vi "FromRepo.vi"(8 "error in":errorcluster, 9 "from repo cluster":T2, 10 "repository in":refnum<class "NISE_CEF_Repository.lvclass">, 11 "engine in":refnum<class "Engine Parent Editor Node.lvclass">) -> (0 "error out":errorcluster, 2 "repository out":refnum<class "NISE_CEF_Repository.lvclass">, 3 "node":T1)   [LabVIEW 2013, in "PL Framework Configuration Tool.lvlib" / "Engine Parent Editor Node.lvclass"]
doc: "Grabs information from the Repo and stores it in the nodes."
uses:
  Engine Parent Editor Node.lvclass
  <vilib>/NI/Configuration Framework/Repository/NISE_CEF_Repository.lvclass
  <vilib>/NI/Configuration Framework/Node/FromRepoCluster.ctl
  <vilib>/NI/Configuration Framework/Node/NodeRef.ctl
  <vilib>/NI/Configuration Framework/Node/NISE_CEF_Node.lvclass
  EngineTags/EngineTags.lvclass
  Engine Mappings/Engine Mappings.lvclass
  TBM Configuration Node/TBM Configuration Node.lvclass
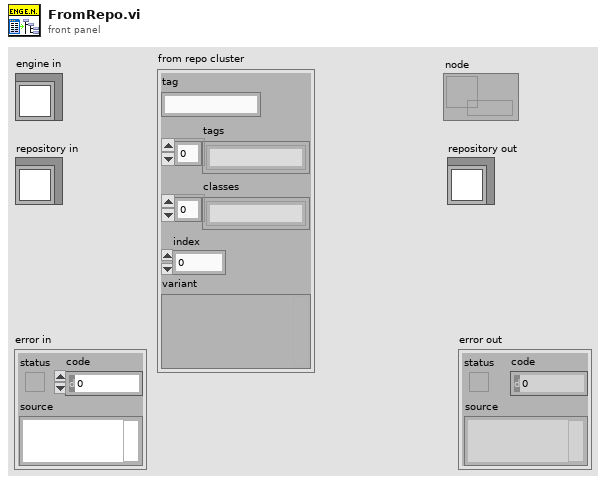
[diagram p1: front panel]
types:
  T1 = typedef "NISE_CEF_Node.lvclass/NodeRef.ctl" = refnum<data-value>
  T2 = typedef "NISE_CEF_Node.lvclass/FromRepoCluster.ctl" = cluster{"tag":string, "tags":string[], "classes":string[], "index":i32, "variant":variant}
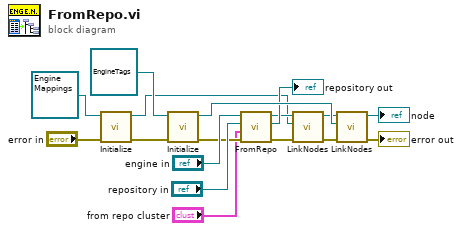
[diagram p0: block diagram]
diagram:
  n1 = call-dynamic "Initialize.vi"("error in"="error in", "node in"=refnum<class "Engine Mappings.lvclass"> refnum ("PL Framework Configuration Tool.lvlib:Engine Mapping Viewer")) -> ("error out"=w6:errorcluster, "data value reference"=w4:T1)  [unwired: 7 in, 1 out]
  n2 = call-dynamic "Initialize.vi"("error in"=w6, "node in"=refnum<class "EngineTags.lvclass"> refnum ("EngineTags.lvclass")) -> ("error out"=w3:errorcluster, "data value reference"=w17:T1)  [unwired: 7 in, 1 out]
  n3 = call-parent "FromRepo.vi"("error in"=w3, "from repo cluster"="from repo cluster", "repository in"="repository in", "node in"="engine in") -> ("error out"=w10:errorcluster, "repository out"=→"repository out":refnum<class "NISE_CEF_Repository.lvclass">, "node"=w9:T1)  [unwired: 5 in]
  n4 = call <vilib>:"LinkNodes.vi"("error in"=w10, "child in"=w4, "parent in"=w9) -> ("error out"=w7:errorcluster, "parent out"=w8:T1)  [unwired: 6 in, 1 out]
  n5 = call <vilib>:"LinkNodes.vi"("error in"=w7, "child in"=w17, "parent in"=w8) -> ("error out"=→"error out":errorcluster, "parent out"=→"node":T1)  [unwired: 6 in, 1 out]
